vi "GetText.vi"(8 "error in":errorcluster, 11 "CEF_Serialize node in":refnum<class "XY Plotter.lvclass">) -> (0 "error out":errorcluster, 1 "additional text":string, 2 "text":string, 3 "CEF_Serialize node out":refnum<class "XY Plotter.lvclass">, 4 "glyph":string)   [LabVIEW 2025, in "XY Plotter.lvlib" / "XY Plotter.lvclass"]
doc: "Returns the text representation of the node used for the tree control.Copyright 2017 National Instruments Corporation\n\nLicensed under the Apache License, Version 2.0 (the \"License\"); you may not use this file except in compliance with the License. You may obtain a copy of the License at http://www.apache.org/licenses/LICENSE-2.0\nUnless required by applicable law or agreed to in writing, software distributed under the License is distributed on an \"AS IS\" BASIS, WITHOUT WARRANTIES OR CONDITIONS OF ANY KIND, either express or implied. See the License for the specific language governing permissions and limitations under the License."
uses:
  XY Plotter.lvclass
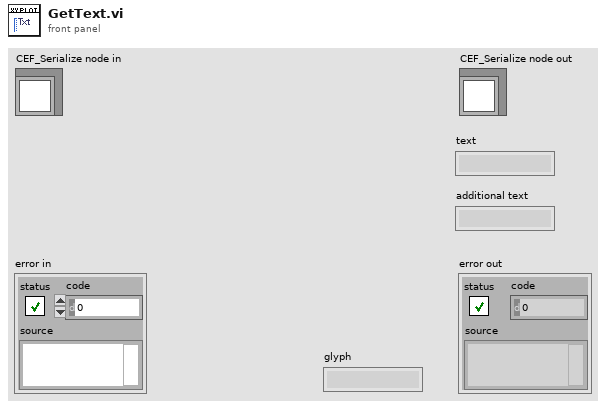
[diagram p1: front panel]
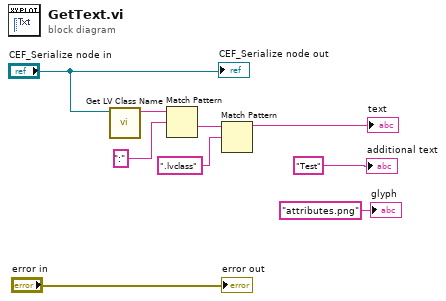
[diagram p0: block diagram]
diagram:
  n1 = call <vilib>:"Get LV Class Name.vi"("object"="CEF_Serialize node in") -> ("class name"=w5:string)  [unwired: 9 in, 1 out]
  n2 = Match Pattern(string=w5, regular expression=":") -> (after substring=w3:string)  [unwired: 1 in, 3 out]
  n3 = Match Pattern(string=w3, regular expression=".lvclass") -> (before substring=→"text":string)  [unwired: 1 in, 3 out]
  "error out" <- "error in"
  "CEF_Serialize node out" <- "CEF_Serialize node in"
  "additional text" <- "Test" ("additional text")
  "glyph" <- "attributes.png" ("glyph")
